vi "Glyph_MouseDown.vi"(6 "Double Click":bool, 8 "error in":errorcluster, 9 "Coords":T5, 10 "CtlRef":refnum<vi>, 11 "Data in":T1={"Class"={"Ants"=refnum, "Layer"=refnum, "Templates"=refnum, "Icon"=refnum, "Glyph"=refnum, "Settings"=refnum, "Tools"=refnum, "History"=refnum}, "Ref"={"Add Layer"=refnum, "Remove Layer"=refnum, "Line Text"=[], "Body Text Spec"=refnum, "DNL_Font"=refnum, "glyph path str"=refnum, "templates path str"=refnum, "Arrow Up"=refnum, "Arrow Down"=refnum, "IE VI Ref"=refnum, "Glyphs tree"=refnum, "Templates tree"=refnum, "Layer Icon Text"=refnum, "Layer Template"=refnum, "Body Text"=refnum, "Search Templates"=refnum, "TextMarker"=refnum, "Tab Control"=refnum, "Search Glyphs"=refnum, "Line Color"=refnum, "DNL_Glyphs []"=refnum, "Fill Color"=refnum, "Tools"=refnum, "Icon"=refnum, "Preview"=refnum, "Ants"=refnum, "Terminals"=refnum, "menu reference"=refnum, "LayerNames"=[], "GlyphLoadAnimation"=refnum, "TemplateLoadAnimation"=refnum, "refreshGlyphs"=refnum, "refreshTemplates"=refnum}, "Support"={"AntsRect"={"left"=0, "top"=0, "right"=0, "bottom"=0}, "Mouse Move Coords"={"Horizontal"=0, "Vertical"=0}, "Mouse Down Coords"={"Horizontal"=0, "Vertical"=0}, "Temp Coord"={"Horizontal"=0, "Vertical"=0}, "Action"=enum."Default", "Edge Color"=4914962, "Fill Color"=16860, "Mouse Down?"=FALSE, "Draft Mode?"=FALSE, "Temp Icon"=bytes[3102], "CTRL Pressed"=FALSE, "Move Selection?"=FALSE, "AntsRect Orig"={"left"=0, "top"=0, "right"=0, "bottom"=0}, "Text"="", "TM Set?"=FALSE, "Mouse inside icon?"=FALSE, "Tool (old value)"=0, "Pencil Move Color"=0, "Swap Colors?"=FALSE, "Shift pressed?"=FALSE}}) -> (0 "error out":errorcluster, 3 "Data out":T1={"Class"={"Ants"=refnum, "Layer"=refnum, "Templates"=refnum, "Icon"=refnum, "Glyph"=refnum, "Settings"=refnum, "Tools"=refnum, "History"=refnum}, "Ref"={"Add Layer"=refnum, "Remove Layer"=refnum, "Line Text"=[], "Body Text Spec"=refnum, "DNL_Font"=refnum, "glyph path str"=refnum, "templates path str"=refnum, "Arrow Up"=refnum, "Arrow Down"=refnum, "IE VI Ref"=refnum, "Glyphs tree"=refnum, "Templates tree"=refnum, "Layer Icon Text"=refnum, "Layer Template"=refnum, "Body Text"=refnum, "Search Templates"=refnum, "TextMarker"=refnum, "Tab Control"=refnum, "Search Glyphs"=refnum, "Line Color"=refnum, "DNL_Glyphs []"=refnum, "Fill Color"=refnum, "Tools"=refnum, "Icon"=refnum, "Preview"=refnum, "Ants"=refnum, "Terminals"=refnum, "menu reference"=refnum, "LayerNames"=[], "GlyphLoadAnimation"=refnum, "TemplateLoadAnimation"=refnum, "refreshGlyphs"=refnum, "refreshTemplates"=refnum}, "Support"={"AntsRect"={"left"=0, "top"=0, "right"=0, "bottom"=0}, "Mouse Move Coords"={"Horizontal"=0, "Vertical"=0}, "Mouse Down Coords"={"Horizontal"=0, "Vertical"=0}, "Temp Coord"={"Horizontal"=0, "Vertical"=0}, "Action"=enum."Default", "Edge Color"=4914962, "Fill Color"=16860, "Mouse Down?"=FALSE, "Draft Mode?"=FALSE, "Temp Icon"=bytes[3102], "CTRL Pressed"=FALSE, "Move Selection?"=FALSE, "AntsRect Orig"={"left"=0, "top"=0, "right"=0, "bottom"=0}, "Text"="", "TM Set?"=FALSE, "Mouse inside icon?"=FALSE, "Tool (old value)"=0, "Pencil Move Color"=0, "Swap Colors?"=FALSE, "Shift pressed?"=FALSE}})   [LabVIEW 2020]
doc: "Performs the actions necessary when there is a Mouse Down event on the Glyph array."
uses:
  Class/Ants/Ants.lvclass
  Class/FakedArray/FakedArray.lvclass
  vi.lib/LabVIEW Icon API/lv_icon/Classes/Icon/Icon.lvclass
  Class/Icon Library/Glyph.lvclass
  Class/Settings/Settings.lvclass
  Class/Tools/Tools Paint.lvclass
  History/History/History.lvclass
  Controls/Tools.ctl
  Controls/SupportClass_Action.ctl
  vi.lib/LabVIEW Icon API/lv_icon/Controls/Graphic.ctl
  History/History.lvlib
  <vilib>/Utility/miscctls.llb/LVPoint32TypeDef.ctl
  vi.lib/LabVIEW Icon API/lv_icon/Controls/IEColor.ctl
  Controls/Support Cluster.ctl
  lv_icon.lvlib
  Controls/References Cluster.ctl
  Controls/IE Classes.ctl
  Controls/Global Data.ctl
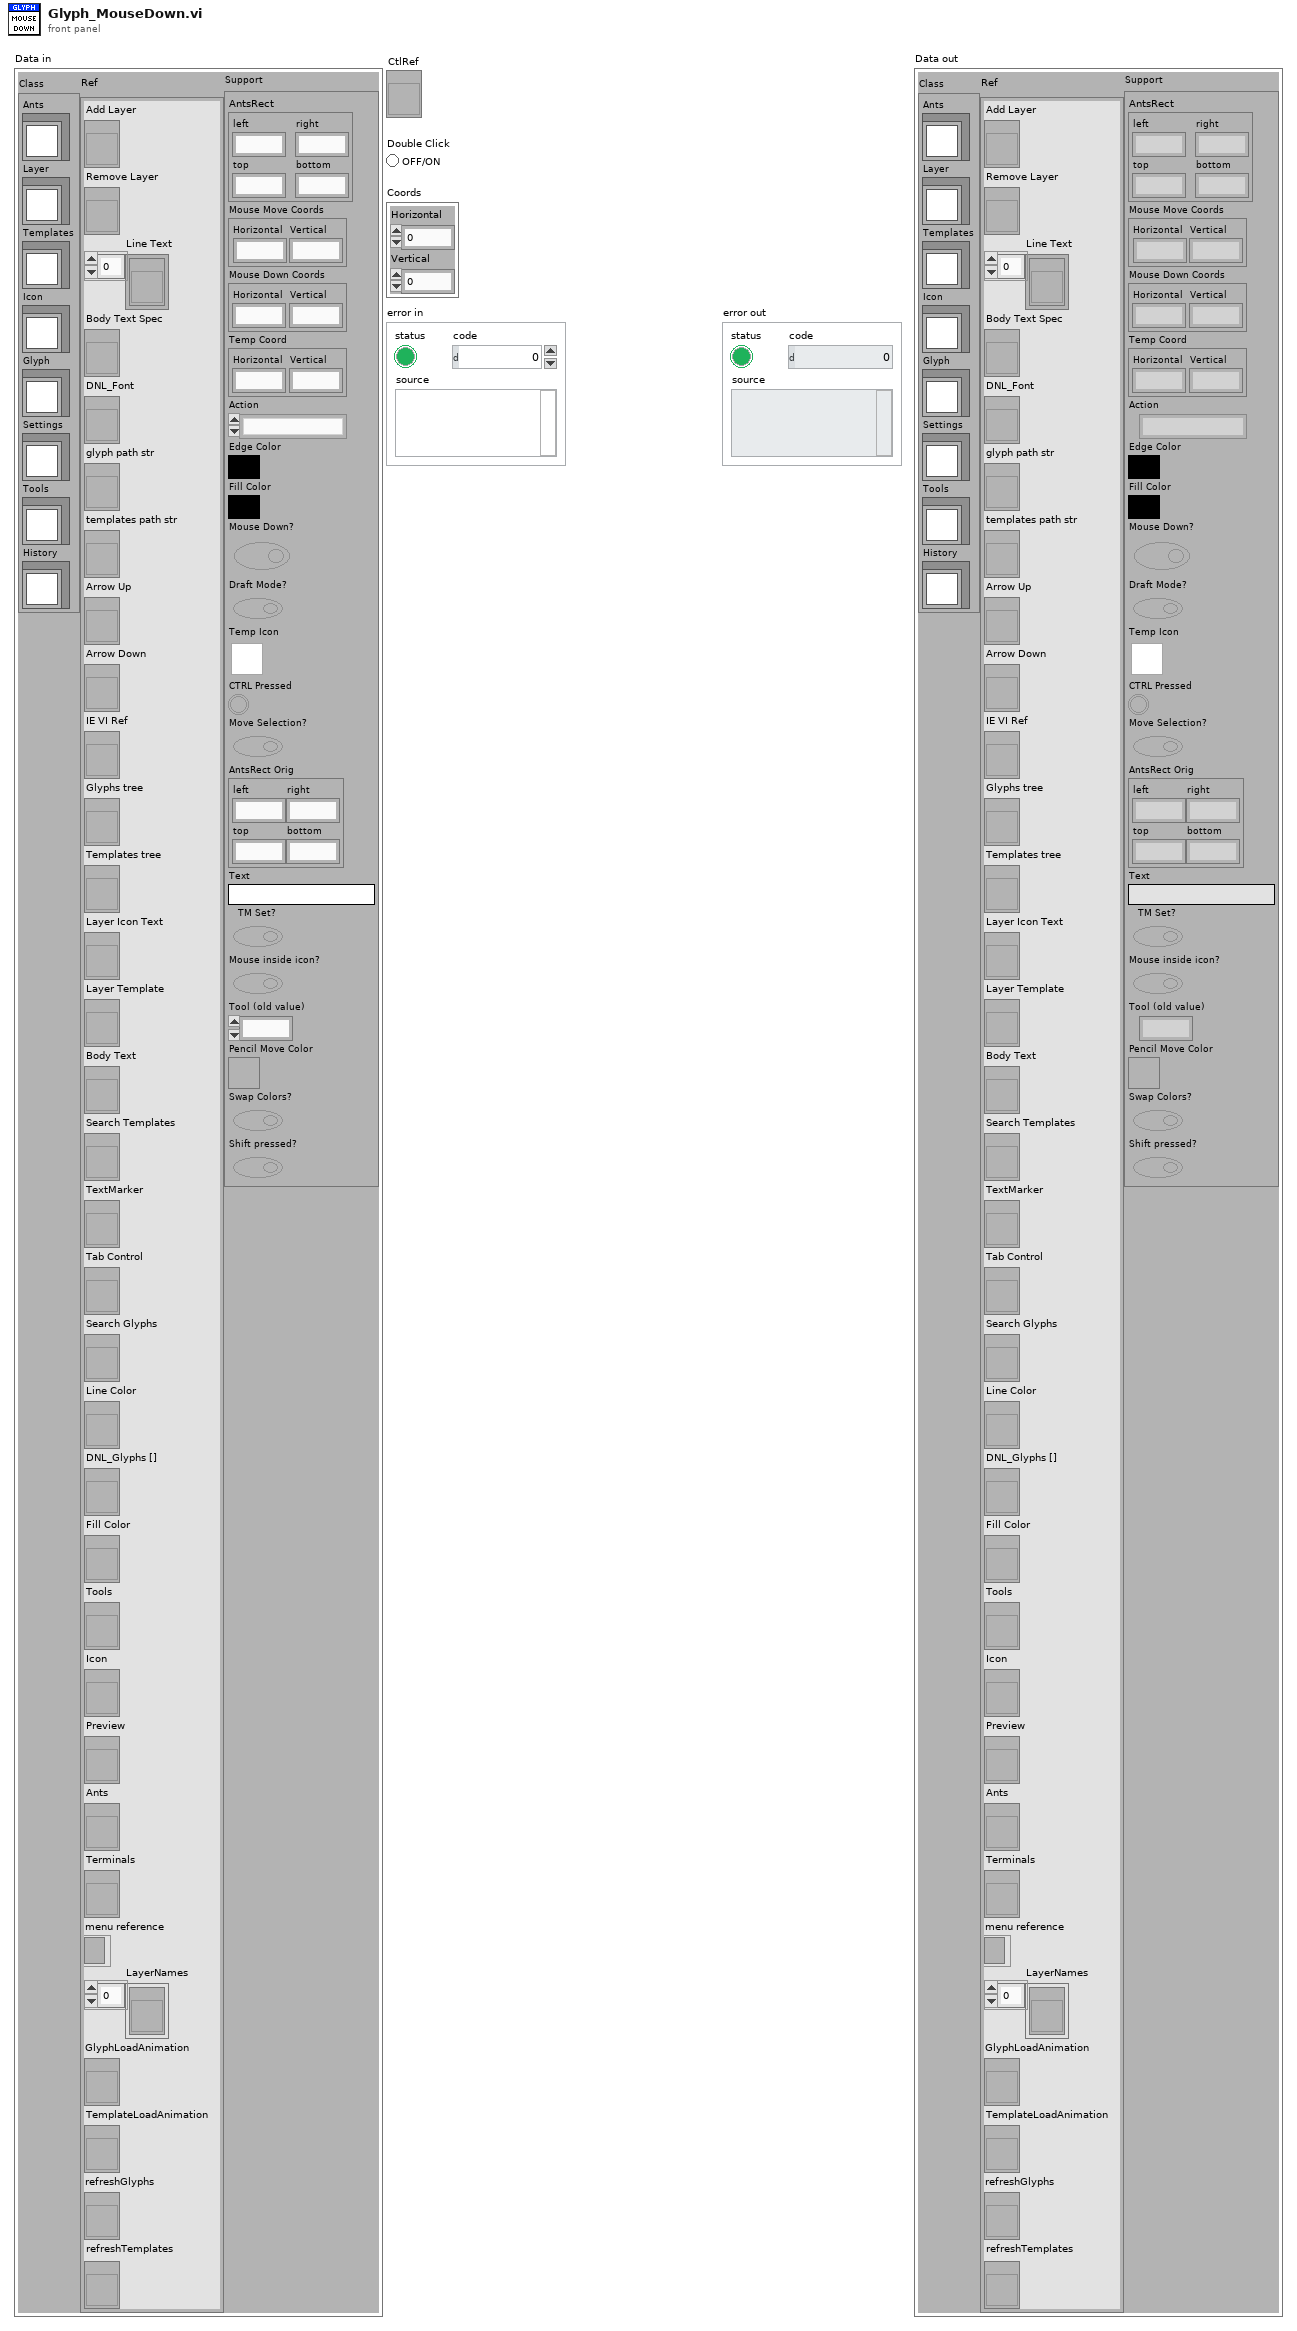
[diagram p1: front panel]
types:
  T1 = typedef "lv_icon.lvlib/Global Data.ctl" = cluster{"Class":T2, "Ref":T3, "Support":T4}
  T2 = typedef "lv_icon.lvlib/IE Classes.ctl" = cluster{"Ants":refnum<class "Ants.lvclass">, "Layer":refnum<class "FakedArray.lvclass">, "Templates":refnum<class "FakedArray.lvclass">, "Icon":refnum<class "Icon.lvclass">, "Glyph":refnum<class "Glyph.lvclass">, "Settings":refnum<class "Settings.lvclass">, "Tools":refnum<class "Tools Paint.lvclass">, "History":refnum<class "History.lvclass">}
  T3 = typedef "lv_icon.lvlib/References Cluster.ctl" = cluster{"Add Layer":refnum<vi>, "Remove Layer":refnum<vi>, "Line Text":refnum<vi>[], "Body Text Spec":refnum<vi>, "DNL_Font":refnum<vi>, "glyph path str":refnum<vi>, "templates path str":refnum<vi>, "Arrow Up":refnum<vi>, "Arrow Down":refnum<vi>, "IE VI Ref":refnum<vi>, "Glyphs tree":refnum<vi>, "Templates tree":refnum<vi>, "Layer Icon Text":refnum<vi>, "Layer Template":refnum<vi>, "Body Text":refnum<vi>, "Search Templates":refnum<vi>, "TextMarker":refnum<vi>, "Tab Control":refnum<vi>, "Search Glyphs":refnum<vi>, "Line Color":refnum<vi>, "DNL_Glyphs []":refnum<vi>, "Fill Color":refnum<vi>, "Tools":refnum<vi>, "Icon":refnum<vi>, "Preview":refnum<vi>, "Ants":refnum<vi>, "Terminals":refnum<vi>, "menu reference":refnum<k9>, "LayerNames":refnum<vi>[], "GlyphLoadAnimation":refnum<vi>, "TemplateLoadAnimation":refnum<vi>, "refreshGlyphs":refnum<vi>, "refreshTemplates":refnum<vi>}
  T4 = typedef "lv_icon.lvlib/Support Cluster.ctl" = cluster{"AntsRect":cluster{"left":i16, "top":i16, "right":i16, "bottom":i16}, "Mouse Move Coords":T5, "Mouse Down Coords":T5, "Temp Coord":T5, "Action":T6, "Edge Color":T7, "Fill Color":T7, "Mouse Down?":bool, "Draft Mode?":bool, "Temp Icon":picture, "CTRL Pressed":bool, "Move Selection?":bool, "AntsRect Orig":cluster{"left":i16, "top":i16, "right":i16, "bottom":i16}, "Text":string, "TM Set?":bool, "Mouse inside icon?":bool, "Tool (old value)":u32, "Pencil Move Color":u32, "Swap Colors?":bool, "Shift pressed?":bool}
  T5 = typedef "LVPoint32TypeDef.ctl" = cluster{"Horizontal":i32, "Vertical":i32}
  T6 = typedef "SupportClass_Action.ctl" = enum16{"Default", "Move Selection", "Glyph Library", "Tool"}
  T7 = typedef "IEColor.ctl" = u32
  T8 = typedef "Graphic.ctl" = cluster{"Rectangle":cluster{"left":i16, "top":i16, "right":i16, "bottom":i16}, "Path":path, "Image":picture, "Filter":string, "FileName":string}
  T9 = typedef "Tools.ctl" = enum32{"Pencil", "Line", "Dropper", "Fill", "Rectangle", "Filled Rectangle", "Ellipse", "Filled Ellipse", "Eraser", "Text", "Select", "Move"}
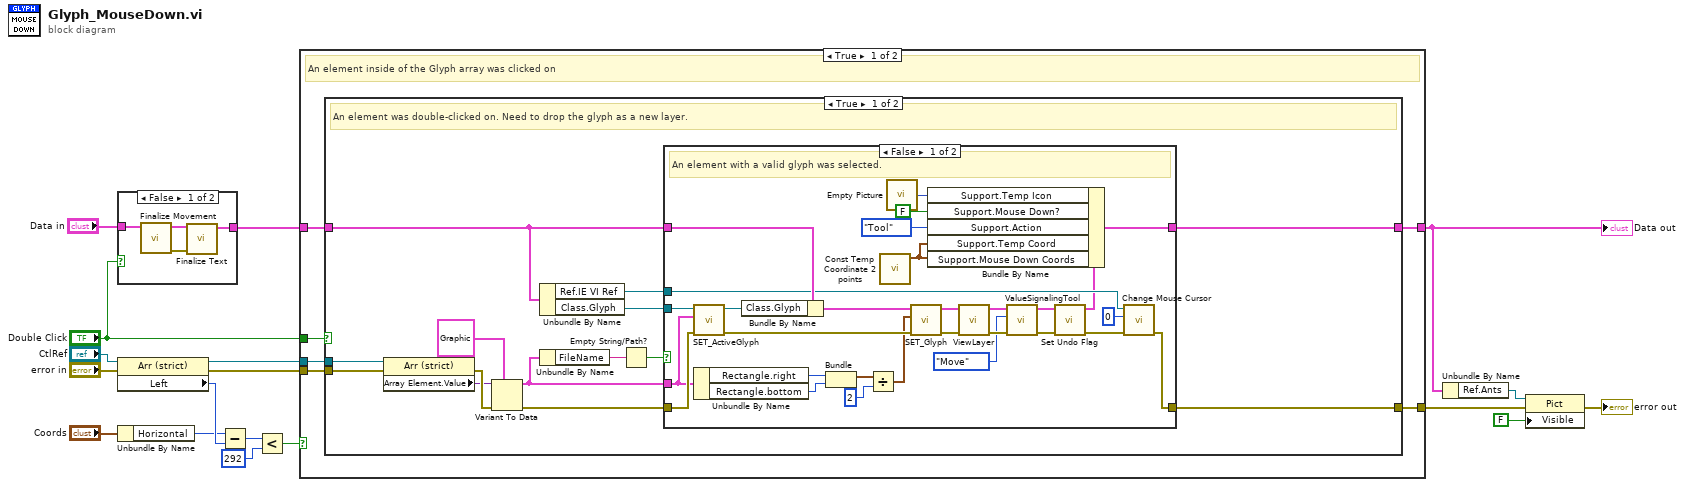
[diagram p0: block diagram]
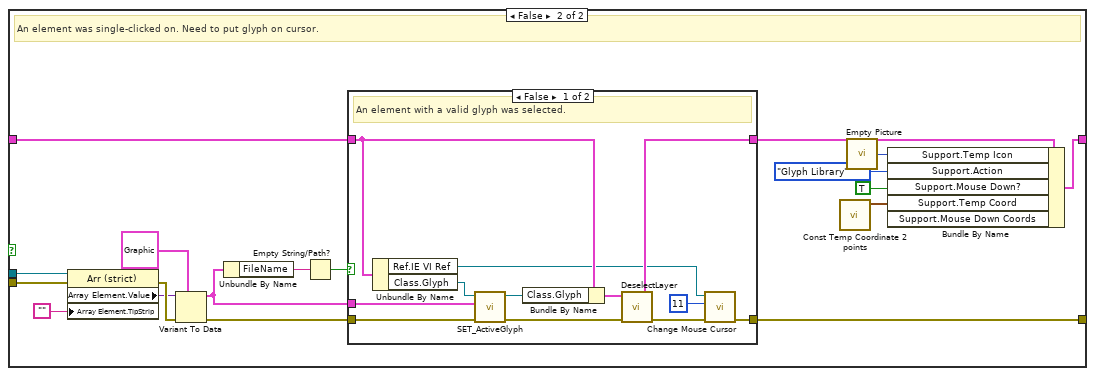
[diagram p4: hidden frame]
diagram:
  n1 = case shown="False" "Double Click" {
    tunnel: "Data in" -> [w21 w23]
    tunnel: [w19 w23] -> w6
    frame False {
      n2 = call "Finalize Movement.vi"("Data in"=w21) -> ("error out"=w22:errorcluster, "Data out"=w20:T1)  [unwired: 2 in, 7 out]
      n3 = call "Finalize Text.vi"("error in (no error)"=w22, "Data in"=w20) -> ("Data out"=w19:T1)  [unwired: 9 out]
    }
    frame True {
    }
  }
  n4 = property class="Arr (strict)"(reference="CtlRef", error in="error in") -> (reference out=w4:refnum<vi>, error out=w15:errorcluster, "Left"=w2:i32)
  n5 = Unbundle By Name("Coords") -> ("Horizontal"=w1:i32)
  n6 = Subtract(x=w1, y=w2) -> (x-y=w3:i32)
  n7 = Less?(x=w3, y=292 ("x")) -> (x < y?=w9:bool)
  n8 = case shown="True" w9 {
    tunnel: w4 -> [w27 _]
    tunnel: w15 -> [w29 w108]
    tunnel: [w28 w108] -> w18
    tunnel: "Double Click" -> [w26 _]
    tunnel: w6 -> [w25 w107]
    tunnel: [w24 w107] -> w5
    frame True {
      # "An element inside of the Glyph array was clicked on"
      n9 = case shown="True" w26 {
        tunnel: w27 -> [w39 w88]
        tunnel: w29 -> [w41 w91]
        tunnel: [w40 w90] -> w28
        tunnel: w25 -> [w35 w80]
        tunnel: [w34 w78] -> w24
        frame True {
          # "An element was double-clicked on. Need to drop the glyph as a new layer."
          n10 = property class="Arr (strict)"(reference=w39, error in=w41) -> (error out=w43:errorcluster, "Array Element.Value"=w38:variant)  [unwired: 1 out]
          n11 = Variant To Data(error in=w43, type=T8 {"Rectangle"={"left"=0, "top"=0, "right"=0, "bottom"=0}, "Path"=path "", "Image"=bytes[0], "Filter"="", "FileName"=""} ("Path & Icon"), Variant=w38) -> (data=w31:T8, error out=w42:errorcluster)
          n12 = Unbundle By Name(w35) -> ("Ref.IE VI Ref"=w33:refnum<vi>, "Class.Glyph"=w36:refnum<class "Glyph.lvclass">)
          n13 = Unbundle By Name(w31) -> ("FileName"=w32:string)
          n14 = Empty String/Path?(string/path=w32) -> (empty?=w30:bool)
          n15 = case shown="False" w30 {
            tunnel: w42 -> [w72 w74]
            tunnel: w36 -> [w56 _]
            tunnel: w35 -> [w54 w73]
            tunnel: [w53 w73] -> w34
            tunnel: w33 -> [w47 _]
            tunnel: [w67 w74] -> w40
            tunnel: w31 -> [w46 _]
            frame False {
              # "An element with a valid glyph was selected."
              n16 = call-dynamic "SET_ActiveGlyph.vi"("error in (no error)"=w72, "Active Glyph"=w46, "Glyph in"=w56) -> ("error out"=w69:errorcluster, "Glyph out"=w55:refnum<class "Glyph.lvclass">)  [unwired: 7 out]
              n17 = Unbundle By Name(w46) -> ("Rectangle.right"=w65:i16, "Rectangle.bottom"=w64:i16)
              n18 = Bundle By Name(cluster=w54, "Class.Glyph"=w55) -> (w52:T1)
              n19 = Bundle("right"=w65, "bottom"=w64) -> (w63:cluster{"right":i16, "bottom":i16})  [unwired: 1 out]
              n20 = Divide(x=w63, y=2) -> (x/y=w61:cluster{"right":dbl, "bottom":dbl})
              n21 = call "Const Temp Coordinate 2 points.vi"() -> ("Const Temp Coordinate"=w57:T5)  [unwired: 11 out]
              n22 = call "Empty Picture"() -> ("empty picture"=w58:picture)
              n23 = call "SET_Glyph.vi"("error in"=w69, "Coordinates"=w61, "Data in"=w52) -> ("error out"=w71:errorcluster, "Data out"=w51:T1)  [unwired: 7 out]
              n24 = call "ViewLayer.vi"("error in (no error)"=w71, "Data in"=w51) -> ("error out"=w70:errorcluster, "Data out"=w49:T1)  [unwired: 3 in, 5 out]
              n25 = call "ValueSignalingTool.vi"("error in (no error)"=w70, "Tools"=Tools."Move", "Data in"=w49) -> ("error out"=w68:errorcluster, "Data out"=w45:T1)  [unwired: 7 out]
              n26 = call "Set Undo Flag.vi"("error in"=w68, "Data in"=w45) -> ("error out"=w66:errorcluster, "Data out"=w44:T1)  [unwired: 8 in]
              n27 = Bundle By Name(cluster=w44, "Support.Temp Icon"=w58, "Support.Mouse Down?"=FALSE ("Mouse Down?"), "Support.Action"=SupportClass_Action."Tool" ("Action"), "Support.Temp Coord"=w57, "Support.Mouse Down Coords"=w57) -> (w53:T1)
              n28 = call "Change Mouse Cursor.vi"("error in (no error)"=w66, "icon"=u16 0, "VI reference (current VI)"=w47) -> ("error out"=w67:errorcluster)  [unwired: 8 out]
            }
            frame True {
            }
          }
        }
        frame False {
          # "An element was single-clicked on. Need to put glyph on cursor."
          n29 = property class="Arr (strict)"(reference=w88, error in=w91, "Array Element.TipStrip"="") -> (error out=w92:errorcluster, "Array Element.Value"=w87:variant)  [unwired: 1 out]
          n30 = Variant To Data(error in=w92, type=T8 {"Rectangle"={"left"=0, "top"=0, "right"=0, "bottom"=0}, "Path"=path "", "Image"=bytes[0], "Filter"="", "FileName"=""} ("Path & Icon 2"), Variant=w87) -> (data=w77:T8, error out=w89:errorcluster)
          n31 = Unbundle By Name(w77) -> ("FileName"=w75:string)
          n32 = Empty String/Path?(string/path=w75) -> (empty?=w76:bool)
          n33 = case shown="False" w76 {
            tunnel: [w103 w106] -> w90
            tunnel: w89 -> [w102 w106]
            tunnel: w80 -> [w99 w105]
            tunnel: [w95 w105] -> w79
            tunnel: w77 -> [w94 _]
            frame False {
              # "An element with a valid glyph was selected."
              n34 = Unbundle By Name(w99) -> ("Ref.IE VI Ref"=w93:refnum<vi>, "Class.Glyph"=w97:refnum<class "Glyph.lvclass">)
              n35 = call-dynamic "SET_ActiveGlyph.vi"("error in (no error)"=w102, "Active Glyph"=w94, "Glyph in"=w97) -> ("error out"=w101:errorcluster, "Glyph out"=w98:refnum<class "Glyph.lvclass">)  [unwired: 7 out]
              n36 = Bundle By Name(cluster=w99, "Class.Glyph"=w98) -> (w96:T1)
              n37 = call "DeselectLayer.vi"("error in (no error)"=w101, "Data in"=w96) -> ("error out"=w104:errorcluster, "Data out"=w95:T1)  [unwired: 8 out]
              n38 = call "Change Mouse Cursor.vi"("error in (no error)"=w104, "icon"=u16 11, "VI reference (current VI)"=w93) -> ("error out"=w103:errorcluster)  [unwired: 8 out]
            }
            frame True {
              # "An invalid glyph was selected."
            }
          }
          n39 = call "Const Temp Coordinate 2 points.vi"() -> ("Const Temp Coordinate"=w82:T5)  [unwired: 11 out]
          n40 = call "Empty Picture"() -> ("empty picture"=w83:picture)
          n41 = Bundle By Name(cluster=w79, "Support.Temp Icon"=w83, "Support.Action"=SupportClass_Action."Glyph Library" ("Action"), "Support.Mouse Down?"=TRUE ("Mouse Down?"), "Support.Temp Coord"=w82, "Support.Mouse Down Coords"=w82) -> (w78:T1)
        }
      }
    }
    frame False {
      # "The scrollbar was clicked on"
    }
  }
  "Data out" <- w5
  n42 = Unbundle By Name(w5) -> ("Ref.Ants"=w10:refnum<vi>)
  n43 = property class="Pict"(reference=w10, error in=w18, "Visible"=FALSE) -> (error out=→"error out":errorcluster)  [unwired: 1 out]
